vi "update Device ID By OPT.vi"(8 "error in (no error)":errorcluster, 10 "Mast Index":i32, 11 "CO3000 in":refnum<class "CO3000.lvclass">) -> (0 "error out":errorcluster, 1 "Mast Available?":bool, 2 "Turn Table Available?":bool, 3 "CO3000 out":refnum<class "CO3000.lvclass">)   [LabVIEW 2023, in "Turn Table and Mast.lvlib" / "CO3000.lvclass"]
uses:
  CO3000.lvclass
  CO3000.lvclass/CO3000.ctl
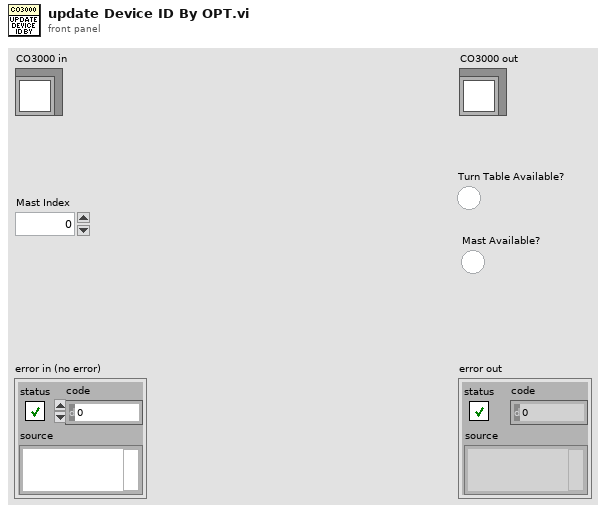
[diagram p1: front panel]
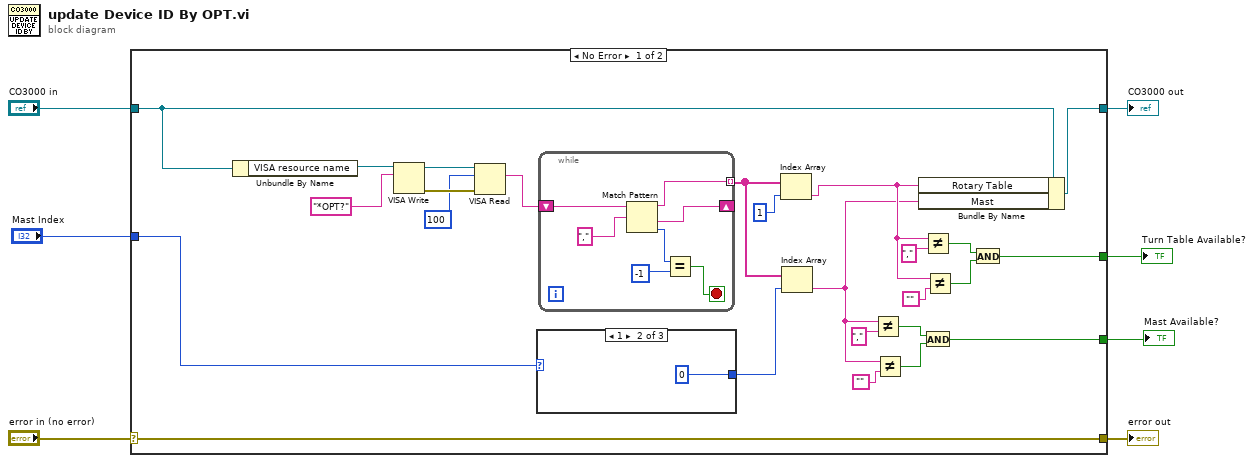
[diagram p0: block diagram]
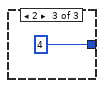
[diagram p3: hidden frame]
diagram:
  n1 = case shown="No Error" "error in (no error)" {
    selector: "error in (no error)" -> [w32 w43]
    tunnel: [w32 w43] -> w6
    tunnel: [w20 w42] -> w4
    tunnel: "CO3000 in" -> [w24 w42]
    tunnel: "Mast Index" -> [w23 _]
    tunnel: [w14 _] -> w2
    tunnel: [w8 _] -> w1
    frame No Error {
      n2 = Unbundle By Name(w24) -> ("VISA resource name"=w31:refnum<visa-resource-name>)
      n3 = VISA Write(VISA resource name=w31, write buffer="*OPT?") -> (VISA resource name out=w29:refnum<visa-resource-name>, error out=w28:errorcluster)  [unwired: 1 in, 1 out]
      n4 = VISA Read(VISA resource name=w29, byte count=u32 100, error in (no error)=w28) -> (read buffer=w26:string)  [unwired: 3 out]
      n5 = case shown="1" w23 {
        tunnel: [_ 0 ("index") 4 ("index")] -> w21
        frame 0, Default {
        }
        frame 1 {
        }
        frame 2 {
        }
      }
      n6 = while {
        shift-right: [w39] -> _
        shift-left: w26 -> [w41]
        tunnel: [w38] -> w22 mode=indexing
        stop <- w35 stop-if-true
        n7 = Match Pattern(string=w41, regular expression=",") -> (before substring=w38:string, after substring=w39:string, offset past match=w37:i32)  [unwired: 1 in, 1 out]
        n8 = Equal?(x=w37, y=-1) -> (x = y?=w35:bool)
      }
      n9 = Index Array(array=w22, index=1) -> (element=w18:string)
      n10 = Index Array(array=w22, index=w21) -> (element=w9:string)
      n11 = Not Equal?(x=w9, y=",") -> (x != y?=w12:bool)
      n12 = Not Equal?(x=w9, y="") -> (x != y?=w13:bool)
      n13 = Bundle By Name(cluster=w24, "Rotary Table"=w18, "Mast"=w9) -> (w20:refnum<class "CO3000.lvclass">)
      n14 = Not Equal?(x=w18, y=",") -> (x != y?=w16:bool)
      n15 = And(x=w12, y=w13) -> (x .and. y?=w8:bool)
      n16 = Not Equal?(x=w18, y="") -> (x != y?=w15:bool)
      n17 = And(x=w16, y=w15) -> (x .and. y?=w14:bool)
    }
    frame Error {
    }
  }
  "error out" <- w6
  "CO3000 out" <- w4
  "Turn Table Available?" <- w2
  "Mast Available?" <- w1
